vi "Get Library Path.vi"() -> (0 "Path":path)   [LabVIEW 2020, in "PV Access.lvlib"]
uses:
  PV Access.lvlib
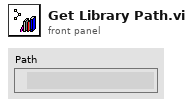
[diagram p1: front panel]
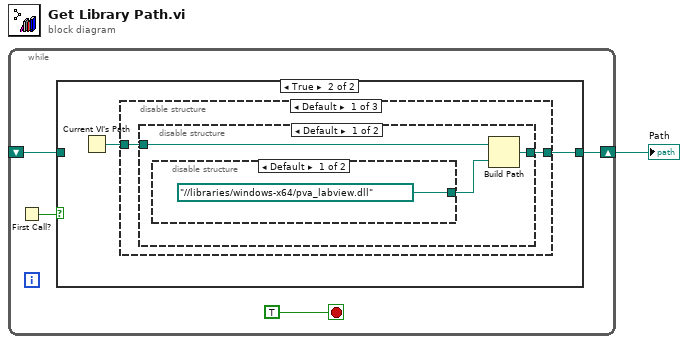
[diagram p0: block diagram]
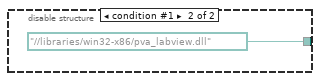
[diagram p3: hidden frame]
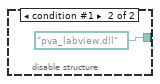
[diagram p4: hidden frame]
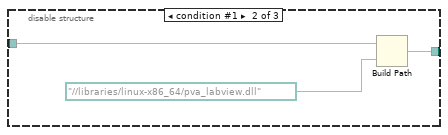
[diagram p5: hidden frame]
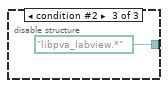
[diagram p6: hidden frame]
diagram:
  n1 = while {
    shift-right: [w5] -> w1
    shift-left: _ -> [w3]
    stop <- TRUE stop-if-true
    n2 = First Call?() -> (First Call?: T/F=w2:bool)
    n3 = case shown="True" w2 {
      tunnel: [w6 w8] -> w5
      tunnel: w3 -> [w6 _]
      frame False {
      }
      frame True {
        n4 = Current VI's Path() -> (path=w7:path)
        n5 = disable-structure shown="Default" {
          disable-tunnel: w7 -> [w9 w17 _]
          disable-tunnel: [w10 w19 path "libpva_labview.*" ("appended path")] -> w8
          frame condition #0 (active) {
            n6 = disable-structure shown="Default" {
              disable-tunnel: [w13 path "pva_labview.dll"] -> w10
              disable-tunnel: w9 -> [w11 _]
              frame condition #0 (active) {
                n7 = disable-structure shown="Default" {
                  disable-tunnel: [path "../../libraries/windows-x64/pva_labview.dll" ("Path") path "../../libraries/win32-x86/pva_labview.dll" ("Path")] -> w12
                  frame condition #0 (active) {
                  }
                  frame condition #1 {
                  }
                }
                n8 = Build Path(base path=w11, name or relative path=w12) -> (appended path=w13:path)
              }
              frame condition #1 {
              }
            }
          }
          frame condition #1 {
            n9 = Build Path(base path=w17, name or relative path=path "../../libraries/linux-x86_64/pva_labview.dll" ("Path")) -> (appended path=w19:path)
          }
          frame condition #2 {
          }
        }
      }
    }
  }
  "Path" <- w1
